vi "RemoteVI Route Request.vi"(0 "path":string, 5 "upgrade request?":bool, 7 "cross origin?":bool, 9 "max clients reached?":bool, 11 "token ok?":bool) -> (4 "status":u16, 6 "page?":bool)   [LabVIEW 2020, in "RemoteVI.lvlib"]
doc: "Decides the HTTP status of a request from its path (docs\\protocol.md section 1): / and /index.html give 200 (page? TRUE); both these and /ws give 403 when token ok? is FALSE (no or a wrong access token, docs\\security.md); /ws gives 426 without a WebSocket upgrade, 403 when the request is cross-origin, 503 when max clients reached? is TRUE, and otherwise 101 (switch to WebSocket); any other path gives 404. Pure. Used by RemoteVI Handle Connection.vi."
uses:
  RemoteVI.lvlib
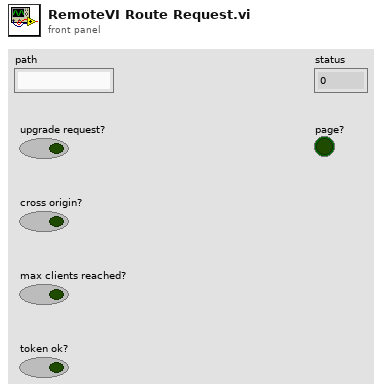
[diagram p1: front panel]
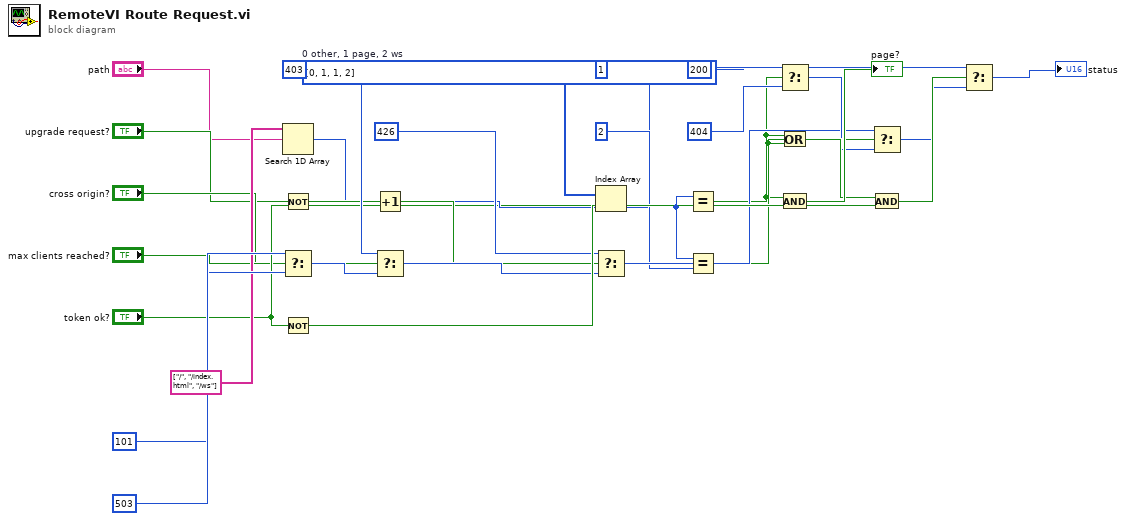
[diagram p0: block diagram]
diagram:
  w18 = u16 403
  w9 = i32[] [0, 1, 1, 2]  # 0 other, 1 page, 2 ws
  n1 = Search 1D Array(1D array=string[] ["/", "/index.html", "/ws"], element="path") -> (index of element=w7:i32)  [unwired: 1 in]
  n2 = Not(x="upgrade request?") -> (.not. x?=w15:bool)
  n3 = Select(t=u16 503, s="max clients reached?", f=u16 101) -> (s? t:f=w22:u16)
  n4 = Not(x="token ok?") -> (.not. x?=w28:bool)
  n5 = Increment(x=w7) -> (x+1=w8:i32)
  n6 = Select(t=w18, s="cross origin?", f=w22) -> (s? t:f=w23:u16)
  n7 = Index Array(array=w9, index=w8) -> (element=w10:i32)
  n8 = Select(t=u16 426, s=w15, f=w23) -> (s? t:f=w24:u16)
  n9 = Equal?(x=w10, y=1) -> (x = y?=w13:bool)
  n10 = Equal?(x=w10, y=2) -> (x = y?=w14:bool)
  n11 = Select(t=u16 200, s=w13, f=u16 404) -> (s? t:f=w25:u16)
  n12 = Or(x=w13, y=w14) -> (x .or. y?=w27:bool)
  n13 = And(x=w13, y="token ok?") -> (x .and. y?=→"page?":bool)
  n14 = Select(t=w24, s=w14, f=w25) -> (s? t:f=w26:u16)
  n15 = And(x=w27, y=w28) -> (x .and. y?=w29:bool)
  n16 = Select(t=w18, s=w29, f=w26) -> (s? t:f=→"status":u16)
